vi "Get Block Diagram.vi"(0 "vi refnum in":refnum<vi>, 1 "error in (no error)":errorcluster) -> (2 "Diagram":refnum<vi>, 3 "vi refnum out":refnum<vi>, 4 "error out":errorcluster)   [LabVIEW 2012, in "Scripting Tools.lvlib"]
doc: "Get a reference to the block diagram of a vi"
uses:
  <userlib>/_LAVAcr/Scripting Tools/Scripting Tools.lvlib
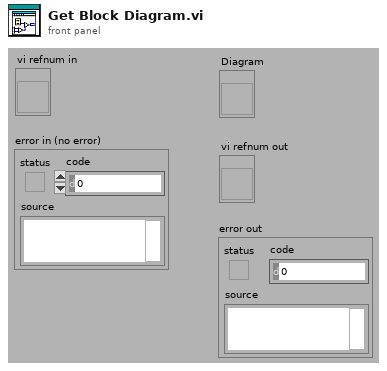
[diagram p1: front panel]
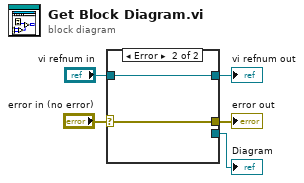
[diagram p0: block diagram]
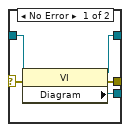
[diagram p2: hidden frame]
diagram:
  n1 = case shown="Error" "error in (no error)" {
    selector: "error in (no error)" -> [w6 w12]
    tunnel: [w10 w11] -> w5
    tunnel: [w9 w12] -> w4
    tunnel: [w8 _] -> w3
    tunnel: "vi refnum in" -> [w7 w11]
    frame No Error {
      n2 = property class="VI"(reference=w7, error in=w6) -> (reference out=w10:refnum<vi>, error out=w9:errorcluster, "Diagram"=w8:refnum<vi>)
    }
    frame Error {
    }
  }
  "vi refnum out" <- w5
  "error out" <- w4
  "Diagram" <- w3
